vi "Example_Lockin.vi"() -> ()   [LabVIEW 2019]
uses:
  Instrument.DAQ/Typedefs/REF.Channel--Cluster--Array.ctl
  Instrument.DAQ/Typedefs/REF.Channel--Cluster.ctl
  Instrument.DAQ/Typedefs/AO.Channel--Cluster--Array.ctl
  Instrument.DAQ/Typedefs/AO.Channel--Cluster.ctl
  Instrument.DAQ/Typedefs/AO.Channel.Function--Enum.ctl
  Instrument.Lockin/Instrument.Lockin.lvclass
  Instrument.DAQ/Instrument.DAQ.lvclass
panel:
  in  "Channels: AO":T1=[{"Enable?"=TRUE, "Channel"=1, "Amplitude"=0.05, "Offset"=0.0, "Frequency"=20.0, "Phase"=0.0, "Function"=enum."sine", "Sweeping?"=FALSE, "Limit AC"=FALSE, "Limit DC?"=FALSE, "Duty Cycle"=FALSE}, {"Enable?"=TRUE, "Channel"=2, "Amplitude"=0.0, "Offset"=0.0, "Frequency"=0.1, "Phase"=0.0, "Function"=enum."sine", "Sweeping?"=FALSE, "Limit AC"=FALSE, "Limit DC?"=FALSE, "Duty Cycle"=FALSE}, {"Enable?"=TRUE, "Channel"=3, "Amplitude"=0.0, "Offset"=0.0, "Frequency"=0.1, "Phase"=0.0, "Function"=enum."sine", "Sweeping?"=FALSE, "Limit AC"=FALSE, "Limit DC?"=FALSE, "Duty Cycle"=FALSE}, {"Enable?"=TRUE, "Channel"=4, "Amplitude"=0.0, "Offset"=0.0, "Frequency"=0.1, "Phase"=0.0, "Function"=enum."sine", "Sweeping?"=FALSE, "Limit AC"=FALSE, "Limit DC?"=FALSE, "Duty Cycle"=FALSE}, {"Enable?"=TRUE, "Channel"=5, "Amplitude"=0.0, "Offset"=0.0, "Frequency"=0.1, "Phase"=0.0, "Function"=enum."sine", "Sweeping?"=FALSE, "Limit AC"=FALSE, "Limit DC?"=FALSE, "Duty Cycle"=FALSE}] {"Phase" format="%#_3g"; "Frequency" min=0.0001 max=200000.0 format="%#_6p"; "Offset" format="%#_6p"; "Amplitude" min=0.0 max=10.0 format="%#_6p"}
  in  "Channels: Lockin":T4=[{"Enable?"=TRUE, "Channel"=1, "Frequency"=20.0, "Phase"=0.0, "TC"=0.1, "Roll-Off"=2}] {"Roll-Off" min=1; "TC" min=0.0001 format="%#_3p"; "Phase" format="%#_3g"; "Frequency" min=0.0001 max=200000.0 format="%#_6p"; "Channel" min=1}
  out "Lockin vs time":cluster{timestamp[], dbl[]}(graph)
  out "Lockin vs parameter":cluster{"Y":dbl[], "Y":dbl[]}(graph)
  in  "step":dbl=0.025
  in  "end":dbl=0.1
  in  "start":dbl
  # "Lockin Example: Lockin\nMake Sure Lockin Program is running!"
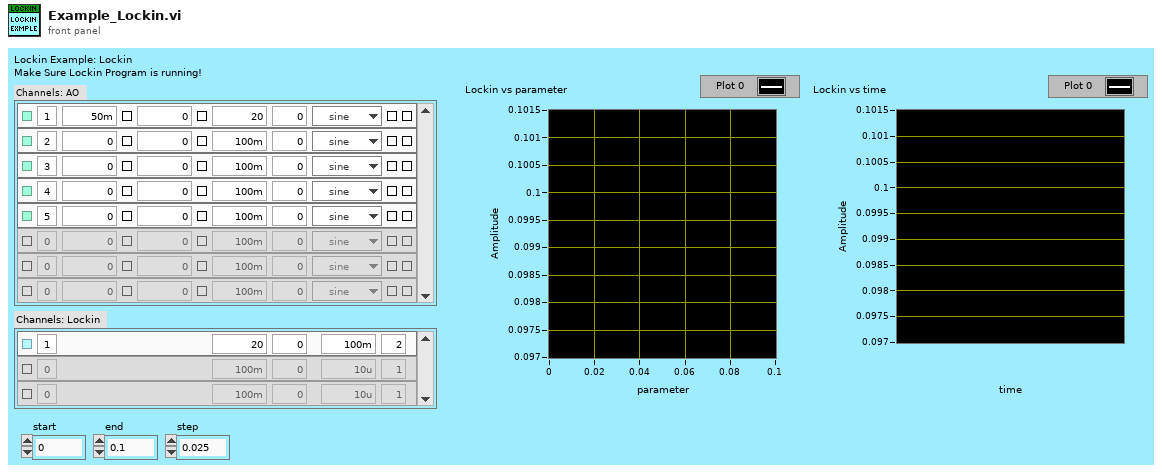
[diagram p1: front panel]
types:
  T1 = typedef "Instrument.Lockin.lvlib/Instrument.DAQ.lvclass/AO.Channel--Cluster--Array.ctl" = T2[]
  T2 = typedef "Instrument.Lockin.lvlib/Instrument.DAQ.lvclass/AO.Channel--Cluster.ctl" = cluster{"Enable?":bool, "Channel":i32, "Amplitude":dbl, "Offset":dbl, "Frequency":dbl, "Phase":dbl, "Function":T3, "Sweeping?":bool, "Limit AC":bool, "Limit DC?":bool, "Duty Cycle":bool}
  T3 = typedef "Instrument.Lockin.lvlib/Instrument.DAQ.lvclass/AO.Channel.Function--Enum.ctl" = enum16{"sine", "square", "triangle", "saw"}
  T4 = typedef "Instrument.Lockin.lvlib/Instrument.DAQ.lvclass/REF.Channel--Cluster--Array.ctl" = T5[]
  T5 = typedef "Instrument.Lockin.lvlib/Instrument.DAQ.lvclass/REF.Channel--Cluster.ctl" = cluster{"Enable?":bool, "Channel":i32, "Frequency":dbl, "Phase":dbl, "TC":dbl, "Roll-Off":i32}
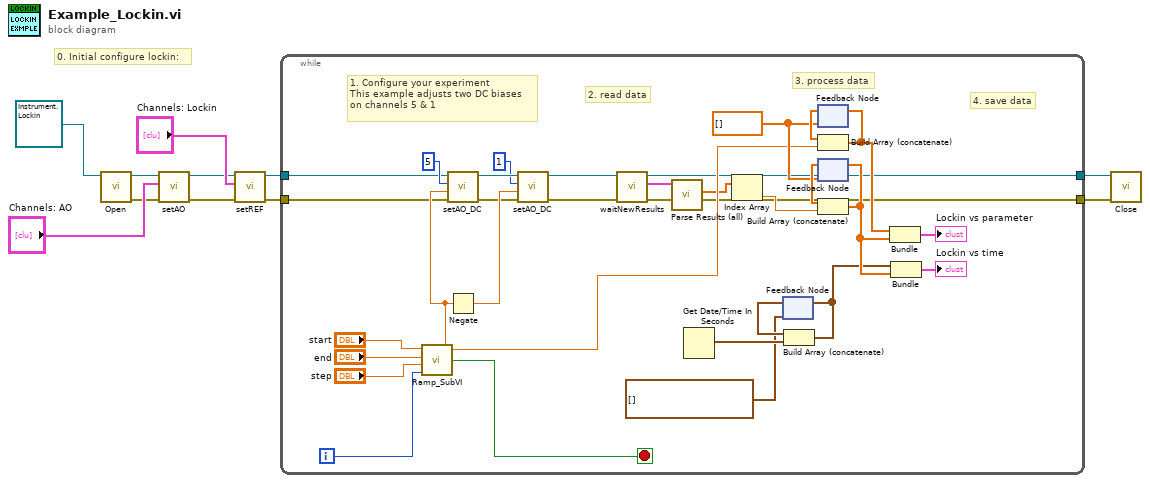
[diagram p0: block diagram]
diagram:
  # "0. Initial configure lockin:"
  n1 = call-dynamic "Open.vi"("Instrument.Lockin in"=refnum<class "Instrument.Lockin.lvclass"> refnum) -> ("error out"=w1:errorcluster, "Instrument.Lockin out"=w3:refnum<class "Instrument.Lockin.lvclass">)  [unwired: 9 in]
  n2 = call-dynamic "setAO.vi"("error in (no error)"=w1, "Channels: AO"="Channels: AO", "Instrument.Lockin in"=w3) -> ("error out"=w9:errorcluster, "Instrument.Lockin out"=w10:refnum<class "Instrument.Lockin.lvclass">)  [unwired: 7 in]
  n3 = call-dynamic "setREF.vi"("error in (no error)"=w9, "Channels: Lockin in"="Channels: Lockin", "Instrument.Lockin in"=w10) -> ("error out"=w7:errorcluster, "Instrument.Lockin out"=w8:refnum<class "Instrument.Lockin.lvclass">)  [unwired: 7 in]
  n4 = while {
    tunnel: w7 -> [w20]
    tunnel: w8 -> [w19]
    tunnel: [w13] -> w5
    tunnel: [w12] -> w4
    i -> [w39]
    stop <- w42 stop-if-true
    w28 = dbl[] []
    # "4. save data"
    # "3. process data"
    # "2. read data"
    # "1. Configure your experiment\nThis example adjusts two DC biases\non channels 5 & 1"
    n5 = call <userlib>:"Ramp_SubVI.vi"("index"=w39, "step"="step", "end"="end", "start"="start") -> ("Stop?"=w42:bool, "Numeric"=w23:dbl)  [unwired: 1 in]
    n6 = call-dynamic "setAO_DC.vi"("error in (no error)"=w20, "DC (V)"=w23, "AO Channel"=5, "Instrument.Lockin in"=w19) -> ("error out"=w21:errorcluster, "Instrument.Lockin out"=w26:refnum<class "Instrument.Lockin.lvclass">)  [unwired: 6 in]
    n7 = Negate(x=w23) -> (-x=w22:dbl)
    n8 = call-dynamic "setAO_DC.vi"("error in (no error)"=w21, "DC (V)"=w22, "AO Channel"=1, "Instrument.Lockin in"=w26) -> ("error out"=w18:errorcluster, "Instrument.Lockin out"=w17:refnum<class "Instrument.Lockin.lvclass">)  [unwired: 6 in]
    n9 = call-dynamic "waitNewResults.vi"("error in (no error)"=w18, "Instrument.Lockin in"=w17) -> ("error out"=w12:errorcluster, "Results (Dictionary)"=w16:cluster{"key":string, "value":dbl}[], "Instrument.Lockin out"=w13:refnum<class "Instrument.Lockin.lvclass">)  [unwired: 7 in]
    n10 = call "Parse Results (all).vi"("Results (Dictionary)"=w16) -> ("Data"=w15:dbl[])  [unwired: 7 in, 3 out]
    n11 = Get Date/Time In Seconds() -> (seconds since 1Jan1904=w31:timestamp)
    n12 = Index Array(array=w15) -> (element=w14:dbl)  [unwired: 1 in]
    n13 = feedback #1(timestamp[] []) -> (w29:timestamp[])
    n14 = Build Array (concatenate)(w29, w31) -> (w30:timestamp[])
    n15 = feedback-in #1(w30) -> ()
    n16 = feedback #2(w28) -> (w33:dbl[])
    n17 = Build Array (concatenate)(w33, w23) -> (w32:dbl[])
    n18 = feedback-in #2(w32) -> ()
    n19 = feedback #3(w28) -> (w35:dbl[])
    n20 = Build Array (concatenate)(w35, w14) -> (w34:dbl[])
    n21 = feedback-in #3(w34) -> ()
    n22 = Bundle(w32, w34) -> (→"Lockin vs parameter":cluster{dbl[], dbl[]})  [unwired: 1 in]
    n23 = Bundle(w30, w34) -> (→"Lockin vs time":cluster{timestamp[], dbl[]})  [unwired: 1 in]
  }
  n24 = call-dynamic "Close.vi"("error in (no error)"=w4, "Instrument.Lockin in"=w5) -> ()  [unwired: 8 in, 2 out]
